vi "macro_ProfiledPIDController_Execute.vi"() -> ()   [LabVIEW 2019, in "Trajectory_Library.lvlib"]
uses:
  Trajectory_Library.lvlib
  ProfiledPIDController_SetPID.vi
  ProfiledPIDController_SetIntegratorRange.vi
  ProfiledPIDController_SetTolerance_PosVel.vi
  ProfiledPIDController_DisableContInput.vi
  ProfiledPIDController_EnableContInput.vi
  ProfiledPIDController_Reset_PosOnly.vi
  ProfiledPIDController_NewPeriod.vi
  ProfiledPIDController_Calculate_Meas_Goal.vi
  ProfiledPIDController_AtGoal.vi
  ProfiledPIDController_AtSetpoint.vi
  ProfiledPIDController_SetConstraints.vi
  PIDController_SetPID.vi
  PIDController_SetIntegratorRange.vi
  PIDController_SetTolerancePandV.vi
  PIDController_DisableContinousInput.vi
  PIDController_EnableContinousInput.vi
  TrapProfState_New.vi
  ProfiledPIDController_Reset.vi
  PIDController_NewPeriod.vi
  <vilib>/Rock Robotics/SystemInterfaces/NetworkCommunication/NetComm_UsageReport_report.vi
  ProfiledPIDController_SetGoal_PosOnly.vi
  ProfiledPIDController_Calculate_Meas.vi
  TrapProfState_Equals.vi
  PIDController_AtSetpoint.vi
  PIDController_Reset.vi
  ProfiledPIDController_SetGoal.vi
  PIDController_Calculate_SP_PV.vi
  TrapProfile_New.vi
  ProfiledPIDController_GetPeriod.vi
  TrapProfile_Calculate.vi
  ControllerUtil_GetModulusError.vi
  PIDController_SetSetpoint.vi
  PIDController_Calculate_PV.vi
  TrapProfile_ShouldFlipAcceleration.vi
  TrapProfile_Direct.vi
  PIDController_GetPeriod.vi
  Globals/Util_LibraryGlobals.vi
panel:
  in  "SP-SetPoint Goal":dbl
  in  "PV-Measurement":dbl
  out "CO-ControlOutput":dbl
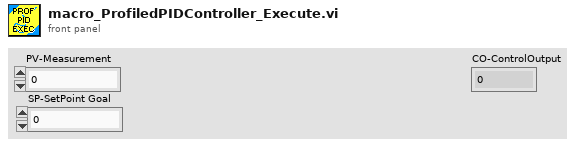
[diagram p1: front panel]
types:
  T1 = typedef "Trajectory_Library.lvlib/PID_TUNING.ctl" = cluster{"Kp":dbl, "Ki":dbl, "Kd":dbl, "MaximumIntegral":dbl, "MinimumIntegral":dbl, "IntegralZone":dbl}
  T2 = typedef "Trajectory_Library.lvlib/PID_ERROR_TOLERANCE.ctl" = cluster{"PositionTolerance":dbl, "VelocityTolerance":dbl}
  T3 = typedef "Trajectory_Library.lvlib/PID_INPUT_LIMITS.ctl" = cluster{"MaxInput":dbl, "MinInput":dbl, "Continuous":bool}
  T4 = typedef "Trajectory_Library.lvlib/TRAPEZOID_PROFILE_CONSTRAINT.ctl" = cluster{"MaxVelocity":dbl, "MaxAcceleration":dbl}
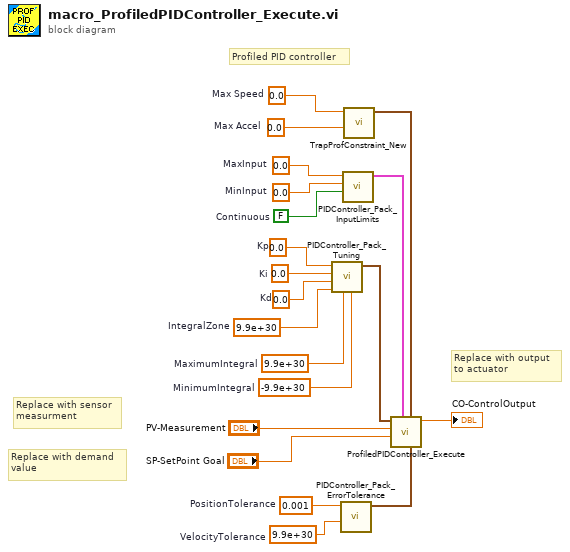
[diagram p0: block diagram]
diagram:
  w1 = 9.9e+30  # IntegralZone
  w5 = 0.001  # PositionTolerance
  w6 = 9.9e+30  # VelocityTolerance
  w8 = 0.0  # Max Speed
  w9 = 0.0  # Max Accel
  w11 = 0.0  # MaxInput
  w12 = 0.0  # MinInput
  w13 = FALSE  # Continuous
  w14 = 0.0  # Kp
  w15 = 0.0  # Ki
  w16 = 0.0  # Kd
  w17 = 9.9e+30  # MaximumIntegral
  w18 = -9.9e+30  # MinimumIntegral
  # "Replace with sensor\nmeasurment"
  # "Replace with demand\nvalue"
  # "Replace with output\nto actuator"
  # "Profiled PID controller"
  n1 = call "PIDController_Pack_Tuning.vi"("MinimumIntegral"=w18, "MaximumIntegral"=w17, "IntegralZone"=w1, "Kd"=w16, "Ki"=w15, "Kp"=w14) -> ("PID Tuning"=w19:T1)  [unwired: 5 in]
  n2 = call "PIDController_Pack_ErrorTolerance.vi"("VelocityTolerance"=w6, "PositionTolerance"=w5) -> ("PID Error Tolerance"=w7:T2)  [unwired: 9 in]
  n3 = call "PIDController_Pack_InputLimits.vi"("Continuous"=w13, "MinInput"=w12, "MaxInput"=w11) -> ("PID Input Limits"=w20:T3)  [unwired: 8 in]
  n4 = call "TrapProfConstraint_New.vi"("Max Accel"=w9, "Max Speed (M/S)"=w8) -> ("TRAPEZOID_PROFILE_CONSTRAINT"=w10:T4)  [unwired: 9 in]
  n5 = call "ProfiledPIDController_Execute.vi"("PID Error Tolerance"=w7, "Constraints"=w10, "PID Input Limits"=w20, "SP-SetPoint Goal"="SP-SetPoint Goal", "PV-Measurement"="PV-Measurement", "PID Tuning"=w19) -> ("CO-ControlOutput"=→"CO-ControlOutput":dbl)  [unwired: 2 in, 3 out]
